vi "getCharactersB_.vi"(8 "error in (no error)":errorcluster, 11 "ocr in":refnum<class "ocr.lvclass">) -> (0 "error out":errorcluster, 3 "ocr out":refnum<class "ocr.lvclass">)   [LabVIEW 2025, in "adsOCR.lvlib" / "ocr.lvclass"]
uses:
  ocr.lvclass
  ocr.lvclass/ocr.ctl
panel:
  in  "noofImgs":i32=1
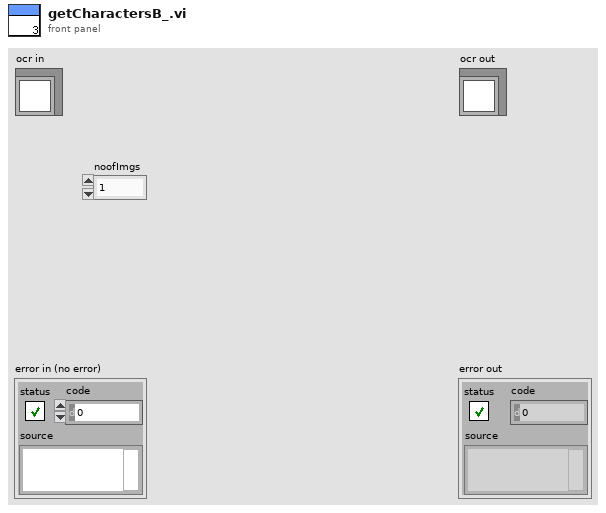
[diagram p1: front panel]
types:
  T1 = typedef "adsOCR.lvlib/ocr.lvclass/TextDecRecResult2L.ctl" = cluster{"imgIdx":i32, "TLx":i32, "TLy":i32, "BRx":i32, "BRy":i32, "angle":sgl, "txtLen":i32}
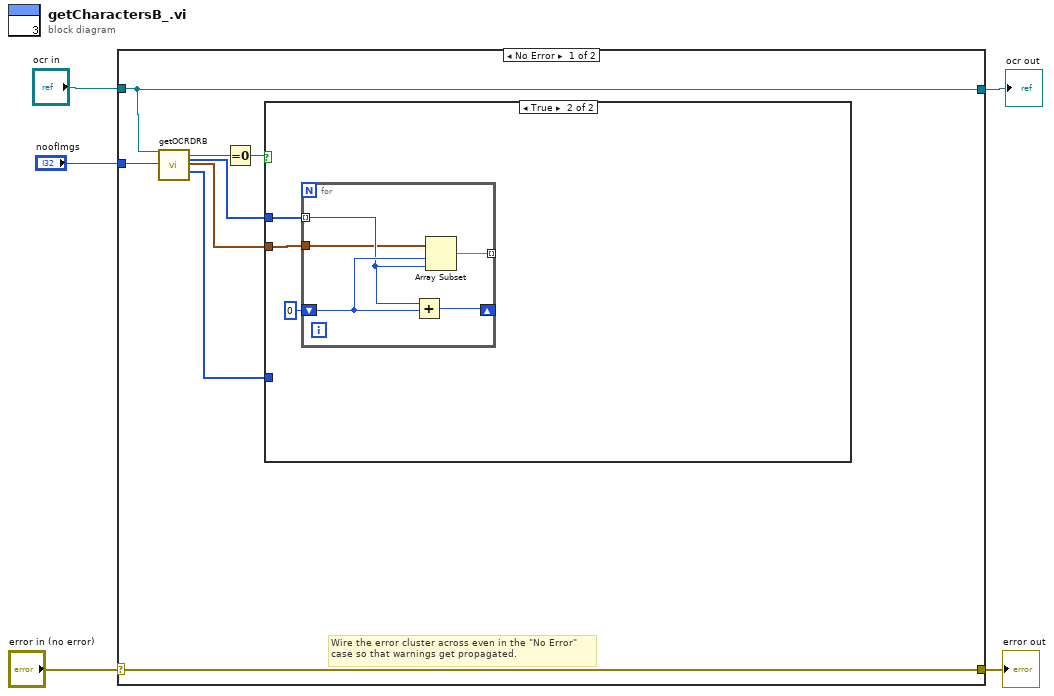
[diagram p0: block diagram]
diagram:
  n1 = case shown="No Error" "error in (no error)" {
    selector: "error in (no error)" -> [w13 w23]
    tunnel: [w13 w23] -> w4
    tunnel: [w11 w22] -> w2
    tunnel: "ocr in" -> [w11 w22]
    tunnel: "noofImgs" -> [w10 _]
    frame No Error {
      # "Wire the error cluster across even in the \"No Error\"\ncase so that warnings get propagated."
      n2 = call-dynamic "getOCRDRB.vi"("ocr in"=w11, "noofImgs"=w10) -> ("succ"=w9:i32, "countsPerImg"=w8:i32[], "TextDecRecResult2L"=w7:T1[], "Chars"=w6:u8[])  [unwired: 19 in, 3 out]
      n3 = Equal To 0?(x=w9) -> (x = 0?=w12:bool)
      n4 = case shown="True" w12 {
        tunnel: w7 -> [_ w16]
        tunnel: w6 -> [_ _]
        tunnel: w8 -> [_ w14]
        frame False {
        }
        frame True {
          n5 = for {
            tunnel: w14 -> [w19] mode=indexing
            tunnel: w16 -> [w18]
            shift-right: [w21] -> _
            shift-left: 0 -> [w20]
            tunnel: [w17] -> _ mode=indexing
            n6 = Add(x=w19, y=w20) -> (x+y=w21:i32)
            n7 = Array Subset(array=w18, index=w20, length=w19) -> (w17:T1[])
          }
        }
      }
    }
    frame Error {
    }
  }
  "error out" <- w4
  "ocr out" <- w2
